vi "open.vi"(8 "error in":errorcluster, 10 "Temporary Folder for Unpacked Files (auto)":path, 11 "Package File Path":path) -> (0 "error out":errorcluster, 3 "PackageFile out":refnum<class "PackageFile.lvclass">)   [LabVIEW 2020, in "vi_package_building_extensions.lvlib" / "PackageFile.lvclass"]
uses:
  PackageFile.lvclass
  PackageFile.lvclass/PackageFile.ctl
  vi_package_building_extensions.lvlib
  <userlib>/_OpenG.lib/file/file.llb/openg_file.lvlib
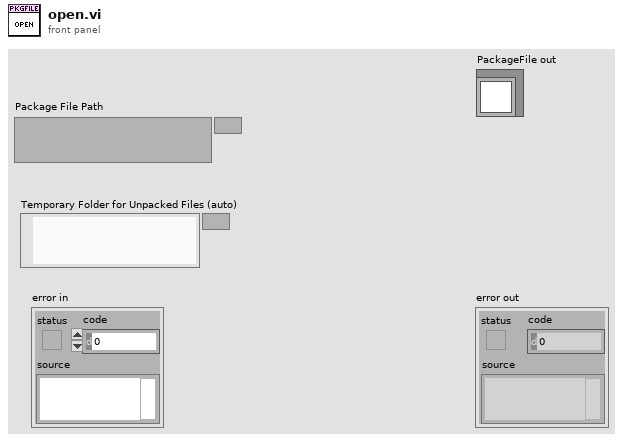
[diagram p1: front panel]
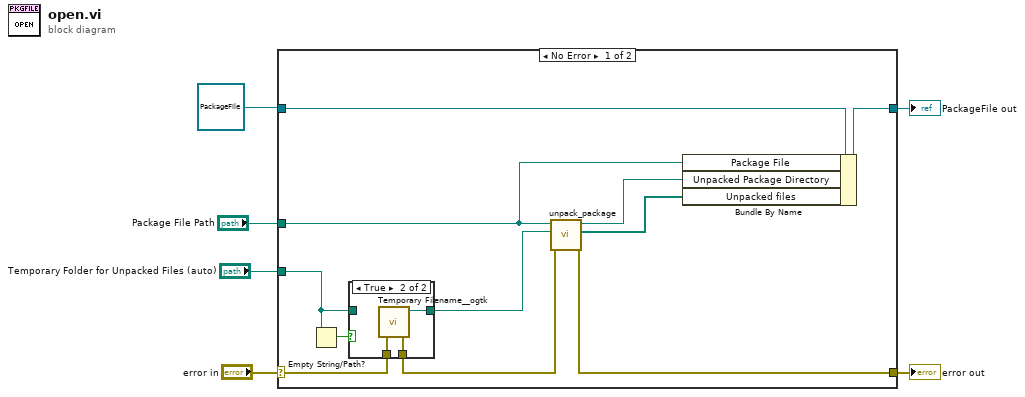
[diagram p0: block diagram]
diagram:
  n1 = case shown="No Error" "error in" {
    selector: "error in" -> [w8 w24]
    tunnel: [w12 w24] -> w5
    tunnel: [w16 w23] -> w3
    tunnel: refnum<class "PackageFile.lvclass"> refnum ("PackageFileEditor in") -> [w17 w23]
    tunnel: "Package File Path" -> [w15 _]
    tunnel: "Temporary Folder for Unpacked Files (auto)" -> [w9 _]
    frame No Error {
      n2 = Empty String/Path?(string/path=w9) -> (empty?=w11:bool)
      n3 = case shown="True" w11 {
        tunnel: [w19 w22] -> w10
        tunnel: w9 -> [w19 _]
        tunnel: w8 -> [w18 w21]
        tunnel: [w18 w20] -> w7
        frame False {
        }
        frame True {
          n4 = call <userlib>:"Temporary Filename__ogtk.vi"("error in (no error)"=w21) -> ("error out"=w20:errorcluster, "file in tmp dir"=w22:path)  [unwired: 5 in]
        }
      }
      n5 = call "unpack_package.vi"("error in (no error)"=w7, "Target directory (same as Package file if empty)"=w10, "Package File"=w15) -> ("error out"=w12:errorcluster, "Unpacked Files"=w13:path[], "Unpacked Package Directory"=w14:path)  [unwired: 6 in]
      n6 = Bundle By Name(cluster=w17, "Package File"=w15, "Unpacked Package Directory"=w14, "Unpacked files"=w13) -> (w16:refnum<class "PackageFile.lvclass">)
    }
    frame Error {
    }
  }
  "error out" <- w5
  "PackageFile out" <- w3
